vi "Autonomous.vi"   [LabVIEW 2025]
doc: "Reefscape 2025 autonomous pattern: dashboard selection followed by a flat sequence. Run the Forward-to-Tag Bordeaux path with Wait, acquire a fresh Limelight AprilTag, turn to its gyro heading if valid, and stop. Autonomous status reports every 20 ms until mode exit."
types:
  T1 = typedef "Command Status Info.ctl" = cluster{"Name":string, "Status":T2, "notifier out":T3}
  T2 = typedef "Completion Status.ctl" = enum16{"Successful", "Aborted", "Incomplete"}
  T3 = typedef "Completion Notifier.ctl" = refnum<notifier>
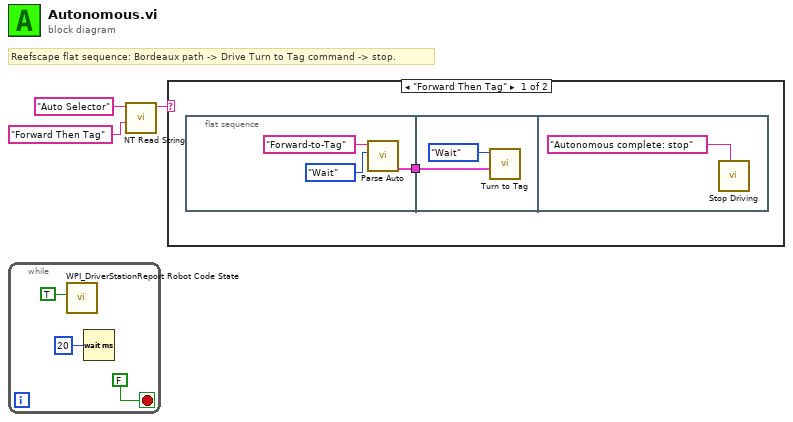
[diagram p0: block diagram]
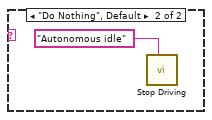
[diagram p2: hidden frame]
diagram:
  # "Reefscape flat sequence: Bordeaux path -> Drive Turn to Tag command -> stop."
  n1 = while {
    stop <- FALSE stop-if-true
    n2 = call <vilib>:"WPI_DriverStationReport Robot Code State.vi"("Autonomous"=TRUE) -> ()  [unwired: 10 in, 1 out]
    n3 = Wait (ms)(milliseconds to wait=u32 20) -> ()  [unwired: 1 out]
  }
  n4 = call <vilib>:"NT Read String.vi"("default value"="Forward Then Tag", "name"="Auto Selector") -> ("value"=w3:string)  [unwired: 7 in, 2 out]
  n5 = case shown="\"Forward Then Tag\"" w3 {
    frame "Forward Then Tag" {
      n6 = flat-sequence {
        tunnel: [w8] -> w7
        tunnel: w7 -> [w11]
        frame #0 {
          n7 = call "Parse Auto.vi"("Synchronization"=enum16{"Start", "Wait"}."Wait", "Name"="Forward-to-Tag") -> ("Command Info Out"=w8:T1)  [unwired: 9 in]
        }
        frame #1 {
          n8 = call "Turn to Tag.vi"("Command Info In"=w11, "Synchronization"=enum16{"Start", "Wait"}."Wait") -> ()  [unwired: 8 in, 2 out]
        }
        frame #2 {
          n9 = call "Stop Driving.vi"("Description"="Autonomous complete: stop") -> ()  [unwired: 10 in, 1 out]
        }
      }
    }
    frame "Do Nothing", Default {
      n10 = call "Stop Driving.vi"("Description"="Autonomous idle") -> ()  [unwired: 10 in, 1 out]
    }
  }
